vi "Copy Files.vi"(8 "error in":errorcluster, 11 "Runner in":refnum<class "Runner.lvclass">) -> (0 "error out":errorcluster, 3 "Runner out":refnum<class "Runner.lvclass">)   [LabVIEW 2026, in "Runner.lvlib" / "Runner.lvclass"]
doc: "Copy VI Template and all dependencies to generated project (amongst others the type definition template)."
uses:
  Runner.lvclass
  Runner.lvclass/Runner.ctl
  Interfaces/ILogger/ILogger Messages/Log Msg/Log Msg.lvclass/Log Msg.ctl
  <vilib>/ActorFramework/Message Enqueuer/Message Enqueuer.lvclass/Message Enqueuer.ctl
  <vilib>/ActorFramework/Message Enqueuer/Enqueue.vi
  Interfaces/ILogger/ILogger Messages/Log Msg/Log Msg.lvclass
  <vilib>/ActorFramework/Message Priority Queue/Priority Enqueue.vi
  <userlib>/_OpenG.lib/file/file.llb/Strip Path Extension - Path__ogtk.vi
  Interfaces/IHash Whitelist Handler/IHash Whitelist Handler.lvclass
  Interfaces/ILV File Creator/ILV File Creator.lvclass
  Interfaces/IFile Manager/IFile Manager.lvclass
  <userlib>/_OpenG.lib/file/file.llb/openg_file.lvlib
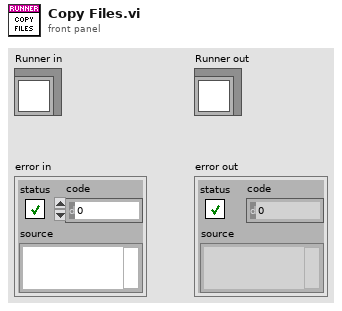
[diagram p1: front panel]
types:
  T1 = typedef "Log Entry--cluster.ctl" = cluster{"Time":timestamp, "Message":string}
  T2 = cluster{i32, "File Path":path, "Paths out":path[]}
  T3 = cluster{i32, "appended path":path, "Paths out":path[]}
  T4 = cluster{i32, "File Path":path, "Paths out":path[]}[]
  T5 = cluster{i32, "appended path":path, "Paths out":path[]}[]
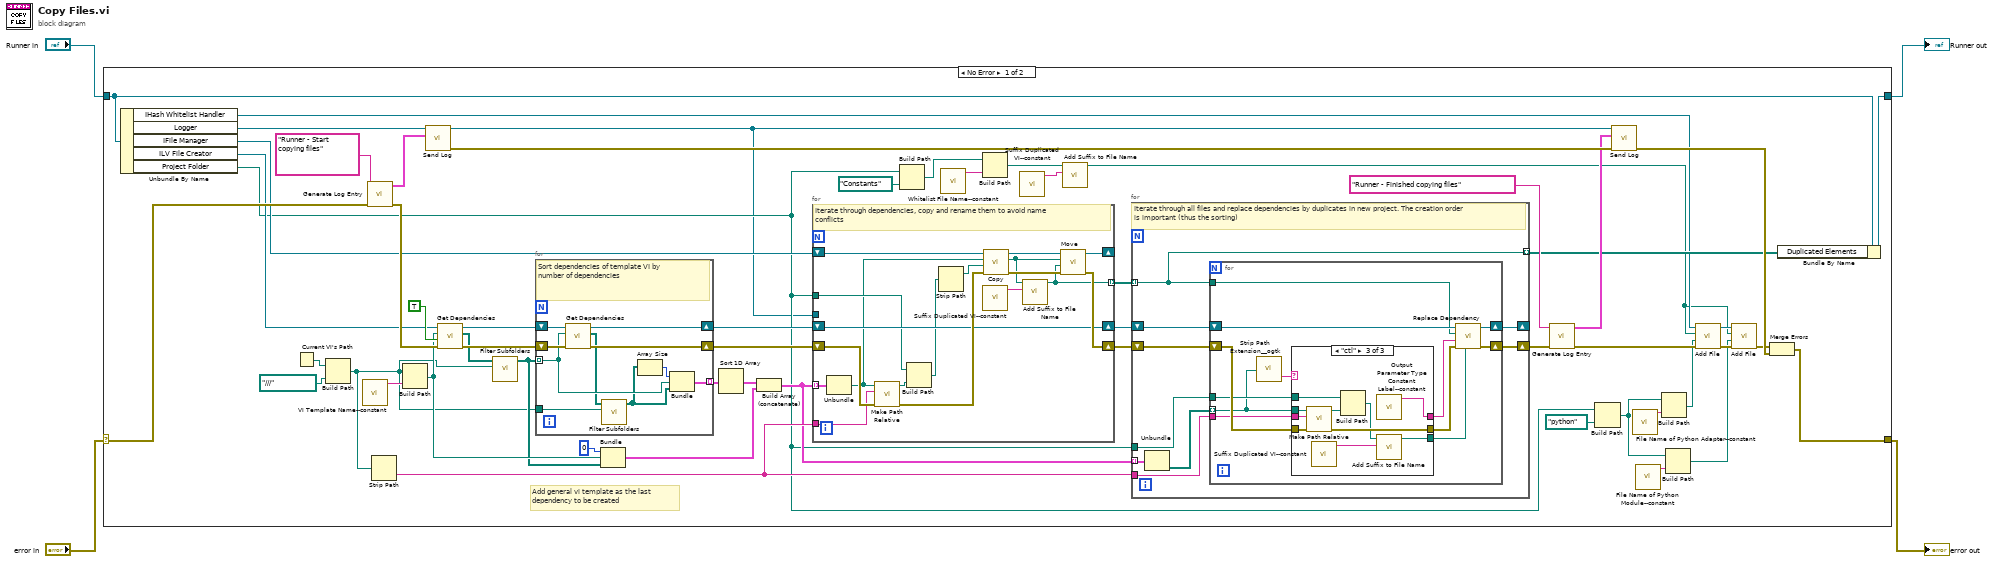
[diagram p0: block diagram]
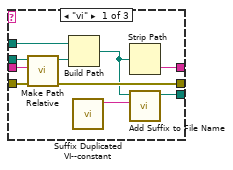
[diagram p2: hidden frame]
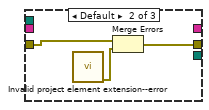
[diagram p3: hidden frame]
diagram:
  n1 = case shown="No Error" "error in" {
    selector: "error in" -> [w53 w134]
    tunnel: [w58 w134] -> w4
    tunnel: "Runner in" -> [w26 w133]
    tunnel: [w24 w133] -> w1
    frame No Error {
      # "Add general vi template as the last\ndependency to be created"
      n2 = Unbundle By Name(w26) -> ("IHash Whitelist Handler"=w21:refnum<class "IHash Whitelist Handler.lvclass">, "Logger"=w48:refnum<class "Message Enqueuer.lvclass">, "IFile Manager"=w38:refnum<class "IFile Manager.lvclass">, "ILV File Creator"=w41:refnum<class "ILV File Creator.lvclass">, "Project Folder"=w19:path)
      n3 = Current VI's Path() -> (path=w43:path)
      n4 = Build Path(base path=w43, name or relative path=path "../../../..") -> (appended path=w8:path)
      n5 = call "VI Template Name--constant.vi"() -> ("VI Template Name"=w27:string)  [unwired: 11 in]
      n6 = call "Generate Log Entry.vi"("error in"=w53, "Message"="Runner - Start copying files") -> ("error out"=w57:errorcluster, "Log Entry"=w47:T1)  [unwired: 8 in]
      n7 = Strip Path(path=w8) -> (name=w35:string)  [unwired: 1 out]
      n8 = Build Path(base path=w8, name or relative path=w27) -> (appended path=w30:path)
      n9 = call "Send Log.vi"("Log Entry"=w47, "Message Enqueuer"=w48) -> ("error out"=w59:errorcluster, "Message Enqueuer out"=w5:refnum<class "Message Enqueuer.lvclass">)  [unwired: 8 in]
      n10 = call-dynamic "Get Dependencies.vi"("error in"=w57, "Entire Hierarchy"=TRUE, "File Path"=w30, "ILV File Creator in"=w41) -> ("error out"=w56:errorcluster, "Dependencies"=w6:path[], "ILV File Creator out"=w39:refnum<class "ILV File Creator.lvclass">)  [unwired: 5 in]
      n11 = call "Filter Subfolders.vi"("Root Path"=w8, "Paths in"=w6) -> ("Paths out"=w29:path[])  [unwired: 9 in]
      n12 = for {
        tunnel: w29 -> [w128] mode=indexing
        tunnel: [w127] -> w40 mode=indexing
        shift-right: [w131] -> w55
        shift-left: w56 -> [w132]
        shift-right: [w126] -> w37
        shift-left: w39 -> [w130]
        tunnel: w8 -> [w124]
        # "Sort dependencies of template VI by number of dependencies"
        n13 = call-dynamic "Get Dependencies.vi"("error in"=w132, "File Path"=w128, "ILV File Creator in"=w130) -> ("error out"=w131:errorcluster, "Dependencies"=w125:path[], "ILV File Creator out"=w126:refnum<class "ILV File Creator.lvclass">)  [unwired: 6 in]
        n14 = call "Filter Subfolders.vi"("Root Path"=w124, "Paths in"=w125) -> ("Paths out"=w123:path[])  [unwired: 9 in]
        n15 = Array Size(array=w123) -> (size(s)=w129:i32)
        n16 = Bundle(w129, "File Path"=w128, "Paths out"=w123) -> (w127:T2)  [unwired: 1 in]
      }
      n17 = Bundle(0, "appended path"=w30, "Paths out"=w29) -> (w28:T3)  [unwired: 1 in]
      n18 = Sort 1D Array(array=w40) -> (sorted array=w36:T4)
      n19 = Build Array (concatenate)(w36, w28) -> (w32:T5)
      n20 = for {
        tunnel: w32 -> [w118] mode=indexing
        tunnel: w35 -> [w108]
        tunnel: w19 -> [w109]
        shift-right: [w111] -> _
        shift-left: w38 -> [w113]
        shift-right: [w112] -> w33
        shift-left: w37 -> [w112]
        shift-right: [w120] -> w54
        shift-left: w55 -> [w119]
        tunnel: [w107] -> w34 mode=indexing
        tunnel: w5 -> [_]
        # "Iterate through dependencies, copy and rename them to avoid name conflicts"
        n21 = Unbundle(w118) -> ("appended path"=w106:path)  [unwired: 2 out]
        n22 = call "Make Path Relative.vi"("error in"=w119, "New Root"=w108, "Absolute Path"=w106) -> ("error out"=w121:errorcluster, "Relative Path"=w117:path)  [unwired: 7 in]
        n23 = Build Path(base path=w109, name or relative path=w117) -> (appended path=w105:path)
        n24 = Strip Path(path=w105) -> (stripped path=w110:path)  [unwired: 1 out]
        n25 = call "Suffix Duplicated VI--constant.vi"() -> ("Suffix Duplicated VI"=w114:string)  [unwired: 11 in]
        n26 = call-dynamic "Copy.vi"("error in"=w121, "Target Folder"=w110, "Source File"=w106, "IFile Manager in"=w113) -> ("error out"=w122:errorcluster, "New Path"=w115:path, "IFile Manager out"=w116:refnum<class "IFile Manager.lvclass">)  [unwired: 5 in]
        n27 = call "Add Suffix to File Name.vi"("Suffix"=w114, "File Path in"=w115) -> ("File Path out"=w107:path)  [unwired: 9 in]
        n28 = call-dynamic "Move.vi"("error in"=w122, "Target"=w107, "Source"=w115, "IFile Manager in"=w116) -> ("error out"=w120:errorcluster, "IFile Manager out"=w111:refnum<class "IFile Manager.lvclass">)  [unwired: 6 in]
      }
      n29 = Build Path(base path=w19, name or relative path=path "Constants") -> (appended path=w17:path)
      n30 = call "Whitelist File Name--constant.vi"() -> ("Whitelist File Name"=w16:string)  [unwired: 11 in]
      n31 = Build Path(base path=w17, name or relative path=w16) -> (appended path=w15:path)
      n32 = call "Suffix Duplicated VI--constant.vi"() -> ("Suffix Duplicated VI"=w14:string)  [unwired: 11 in]
      n33 = call "Add Suffix to File Name.vi"("Suffix"=w14, "File Path in"=w15) -> ("File Path out"=w9:path)  [unwired: 9 in]
      n34 = for {
        tunnel: w32 -> [w67] mode=indexing
        tunnel: w35 -> [w65]
        tunnel: w19 -> [w64]
        tunnel: w34 -> [w61] mode=indexing
        shift-right: [w62] -> _
        shift-left: w33 -> [w63]
        shift-right: [w68] -> w52
        shift-left: w54 -> [w69]
        tunnel: [w61] -> w25 mode=indexing
        # "Iterate through all files and replace dependencies by duplicates in new project. The creation order is important (thus the sorting)"
        n35 = Unbundle(w67) -> ("Paths out"=w66:path[])  [unwired: 2 out]
        n36 = for {
          tunnel: w66 -> [w70] mode=indexing
          shift-right: [w77] -> w62
          shift-left: w63 -> [w78]
          shift-right: [w81] -> w68
          shift-left: w69 -> [w80]
          tunnel: w61 -> [w73]
          tunnel: w64 -> [w71]
          tunnel: w65 -> [w74]
          n37 = call-poly <userlib>:"Strip Path Extension__ogtk.vi"("path"=w70) -> ("extension"=w72:string)  [unwired: 1 out]
          n38 = case shown="\"ctl\"" w72 {
            tunnel: w80 -> [w91 w94 w104]
            tunnel: [w90 w92 w103] -> w79
            tunnel: [w89 _ w95] -> w76
            tunnel: [w87 _ w101] -> w75
            tunnel: w70 -> [w86 _ w100]
            tunnel: w71 -> [w85 _ w99]
            tunnel: w74 -> [w83 _ w97]
            frame "vi" {
              n39 = call "Make Path Relative.vi"("error in"=w91, "New Root"=w83, "Absolute Path"=w86) -> ("error out"=w90:errorcluster, "Relative Path"=w84:path)  [unwired: 7 in]
              n40 = Build Path(base path=w85, name or relative path=w84) -> (appended path=w82:path)
              n41 = call "Suffix Duplicated VI--constant.vi"() -> ("Suffix Duplicated VI"=w88:string)  [unwired: 11 in]
              n42 = Strip Path(path=w82) -> (name=w89:string)  [unwired: 1 out]
              n43 = call "Add Suffix to File Name.vi"("Suffix"=w88, "File Path in"=w82) -> ("File Path out"=w87:path)  [unwired: 9 in]
            }
            frame Default {
              n44 = call "Invalid project element extension--error.vi"() -> ("error out"=w93:errorcluster)  [unwired: 11 in]
              n45 = Merge Errors(w94, w93) -> (w92:errorcluster)
            }
            frame "ctl" {
              n46 = call "Make Path Relative.vi"("error in"=w104, "New Root"=w97, "Absolute Path"=w100) -> ("error out"=w103:errorcluster, "Relative Path"=w98:path)  [unwired: 7 in]
              n47 = call "Suffix Duplicated VI--constant.vi"() -> ("Suffix Duplicated VI"=w102:string)  [unwired: 11 in]
              n48 = Build Path(base path=w99, name or relative path=w98) -> (appended path=w96:path)
              n49 = call "Output Parameter Type Constant Label--constant.vi"() -> ("Output Parameter Type Constant Label"=w95:string)  [unwired: 11 in]
              n50 = call "Add Suffix to File Name.vi"("Suffix"=w102, "File Path in"=w96) -> ("File Path out"=w101:path)  [unwired: 9 in]
            }
          }
          n51 = call-dynamic "Replace Dependency.vi"("New SubVI"=w75, "error in"=w79, "SubVI"=w76, "VI Path"=w73, "ILV File Creator in"=w78) -> ("error out"=w81:errorcluster, "ILV File Creator out"=w77:refnum<class "ILV File Creator.lvclass">)  [unwired: 5 in]
        }
      }
      n52 = call "Generate Log Entry.vi"("error in"=w52, "Message"="Runner - Finished copying files") -> ("error out"=w51:errorcluster, "Log Entry"=w45:T1)  [unwired: 8 in]
      n53 = Build Path(base path=w19, name or relative path=path "python") -> (appended path=w11:path)
      n54 = call "Send Log.vi"("error in (no error)"=w59, "Log Entry"=w45, "Message Enqueuer"=w5) -> ("error out"=w60:errorcluster)  [unwired: 7 in, 1 out]
      n55 = call "File Name of Python Adapter--constant.vi"() -> ("File Name of Python Adapter"=w23:string)  [unwired: 11 in]
      n56 = call "File Name of Python Module--constant.vi"() -> ("File Name of Python Module"=w12:string)  [unwired: 11 in]
      n57 = Build Path(base path=w11, name or relative path=w23) -> (appended path=w20:path)
      n58 = Build Path(base path=w11, name or relative path=w12) -> (appended path=w10:path)
      n59 = call-dynamic "Add File.vi"("error in"=w51, "File Path"=w20, "Whitelist constant"=w9, "IHash Whitelist Handler in"=w21) -> ("error out"=w50:errorcluster, "IHash Whitelist Handler out"=w13:refnum<class "IHash Whitelist Handler.lvclass">)  [unwired: 6 in]
      n60 = call-dynamic "Add File.vi"("error in"=w50, "File Path"=w10, "Whitelist constant"=w9, "IHash Whitelist Handler in"=w13) -> ("error out"=w49:errorcluster)  [unwired: 6 in, 1 out]
      n61 = Merge Errors(w49, w60) -> (w58:errorcluster)
      n62 = Bundle By Name(cluster=w26, "Duplicated Elements"=w25) -> (w24:refnum<class "Runner.lvclass">)
    }
    frame Error {
      # "Pass error without actions."
    }
  }
  "error out" <- w4
  "Runner out" <- w1
